vi "Ref Plots Viewer.vi"() -> ()   [LabVIEW 2020]
uses:
  Typedefs/Ref plot graphs cluster.ctl
  RIG-SPECIFIC FILES/FPGA Refs/FPGA Ref.ctl
  Movement Correction/Typedefs/Reference plots window ctrl refs.ctl
  Typedefs/Save-Load enum.ctl
  Typedefs/fgv_actions.ctl
  Typedefs/Read Write Enum.ctl
  templates/Queue Access FGV/Controls/FGV State Command.ctl
  Global Variables/General Globals.vi
  Globals/gl_Windows Ctrl refs.vi
  <vilib>/Utility/error.llb/Error Cluster From Error Code.vi
  <vilib>/rvi/errors/niLvFpgaAdjustHostInterfaceError.vi
  Global Variables/FPGAstatus_Reference.vi
  <vilib>/rvi/interface/nirviReadWriteControl/nirviReadWriteControl.xnode
  <vilib>/rvi/interface/Simulation/niFpgaSimulationCallBeginRW.vi
  NiFpgaLv.dll
panel:
  in  "Auto reset":bool
  out "Actual refresh rate (ms)":u32
  in  "Initiate reset":bool
  in  "Lower limits [um]":dbl=-115.0
  in  "Upper limits [um]":dbl=115.0
  out "L1 Time":u32
  out "L2 Time":u32
  out "# pending insert":i32
  out "# pending remove":i32
  out "RESTART MC":bool
  out "Reset Transition Status":T1(ring)
  out "Status":T2(ring)
  out "Graph Updating":bool
  in  "Ref image thresholding":cluster{"Numeric":dbl, "Numeric":dbl}(slide)={"Numeric"=0.0, "Numeric"=819.0} scale=0.0..4095.0
  out "Test GraphData Path":path
  in  "Append Date-Time":bool
  in  "Append file name":string
  out "MC Data Save ON":bool
  in  "Save MC Data":bool
  in  "Nth Frame":u16=11 min=10 step=10
  out "end of trial":i16(graph)
  in  "Frames":i16=1
  out "FPGA VI Reference Out":T3
  in  "Maximum Value":i32=4095
  in  "Minimum Value":i32
  out "Ref Image":T4(plugin-control)
  out "background_mc":bool
  out "bgsm_state":T5(ring)
  out "Acquire MC BG":bool
  out "rec_on_bg":bool
  out "aq state":T6(ring)
  in  "Acquisition completed":bool
  out "Stop (ind)":bool
  out "error":errorcluster
  in  "Snapshot file path":path caption="Snapshot file path (data is appended if same file used)"
  in  "Buffer Size":i32=5000 min=5 max=10000 step=100
  in  "Refresh rate (ms)":u32=500 min=10 step=10
  in  "Snapshot":bool
  in  "Reset Graphs":bool
  out "Graphs cluster":T7
  # "(during live imaging)"
  # "12"
  # "2"
  # "0"
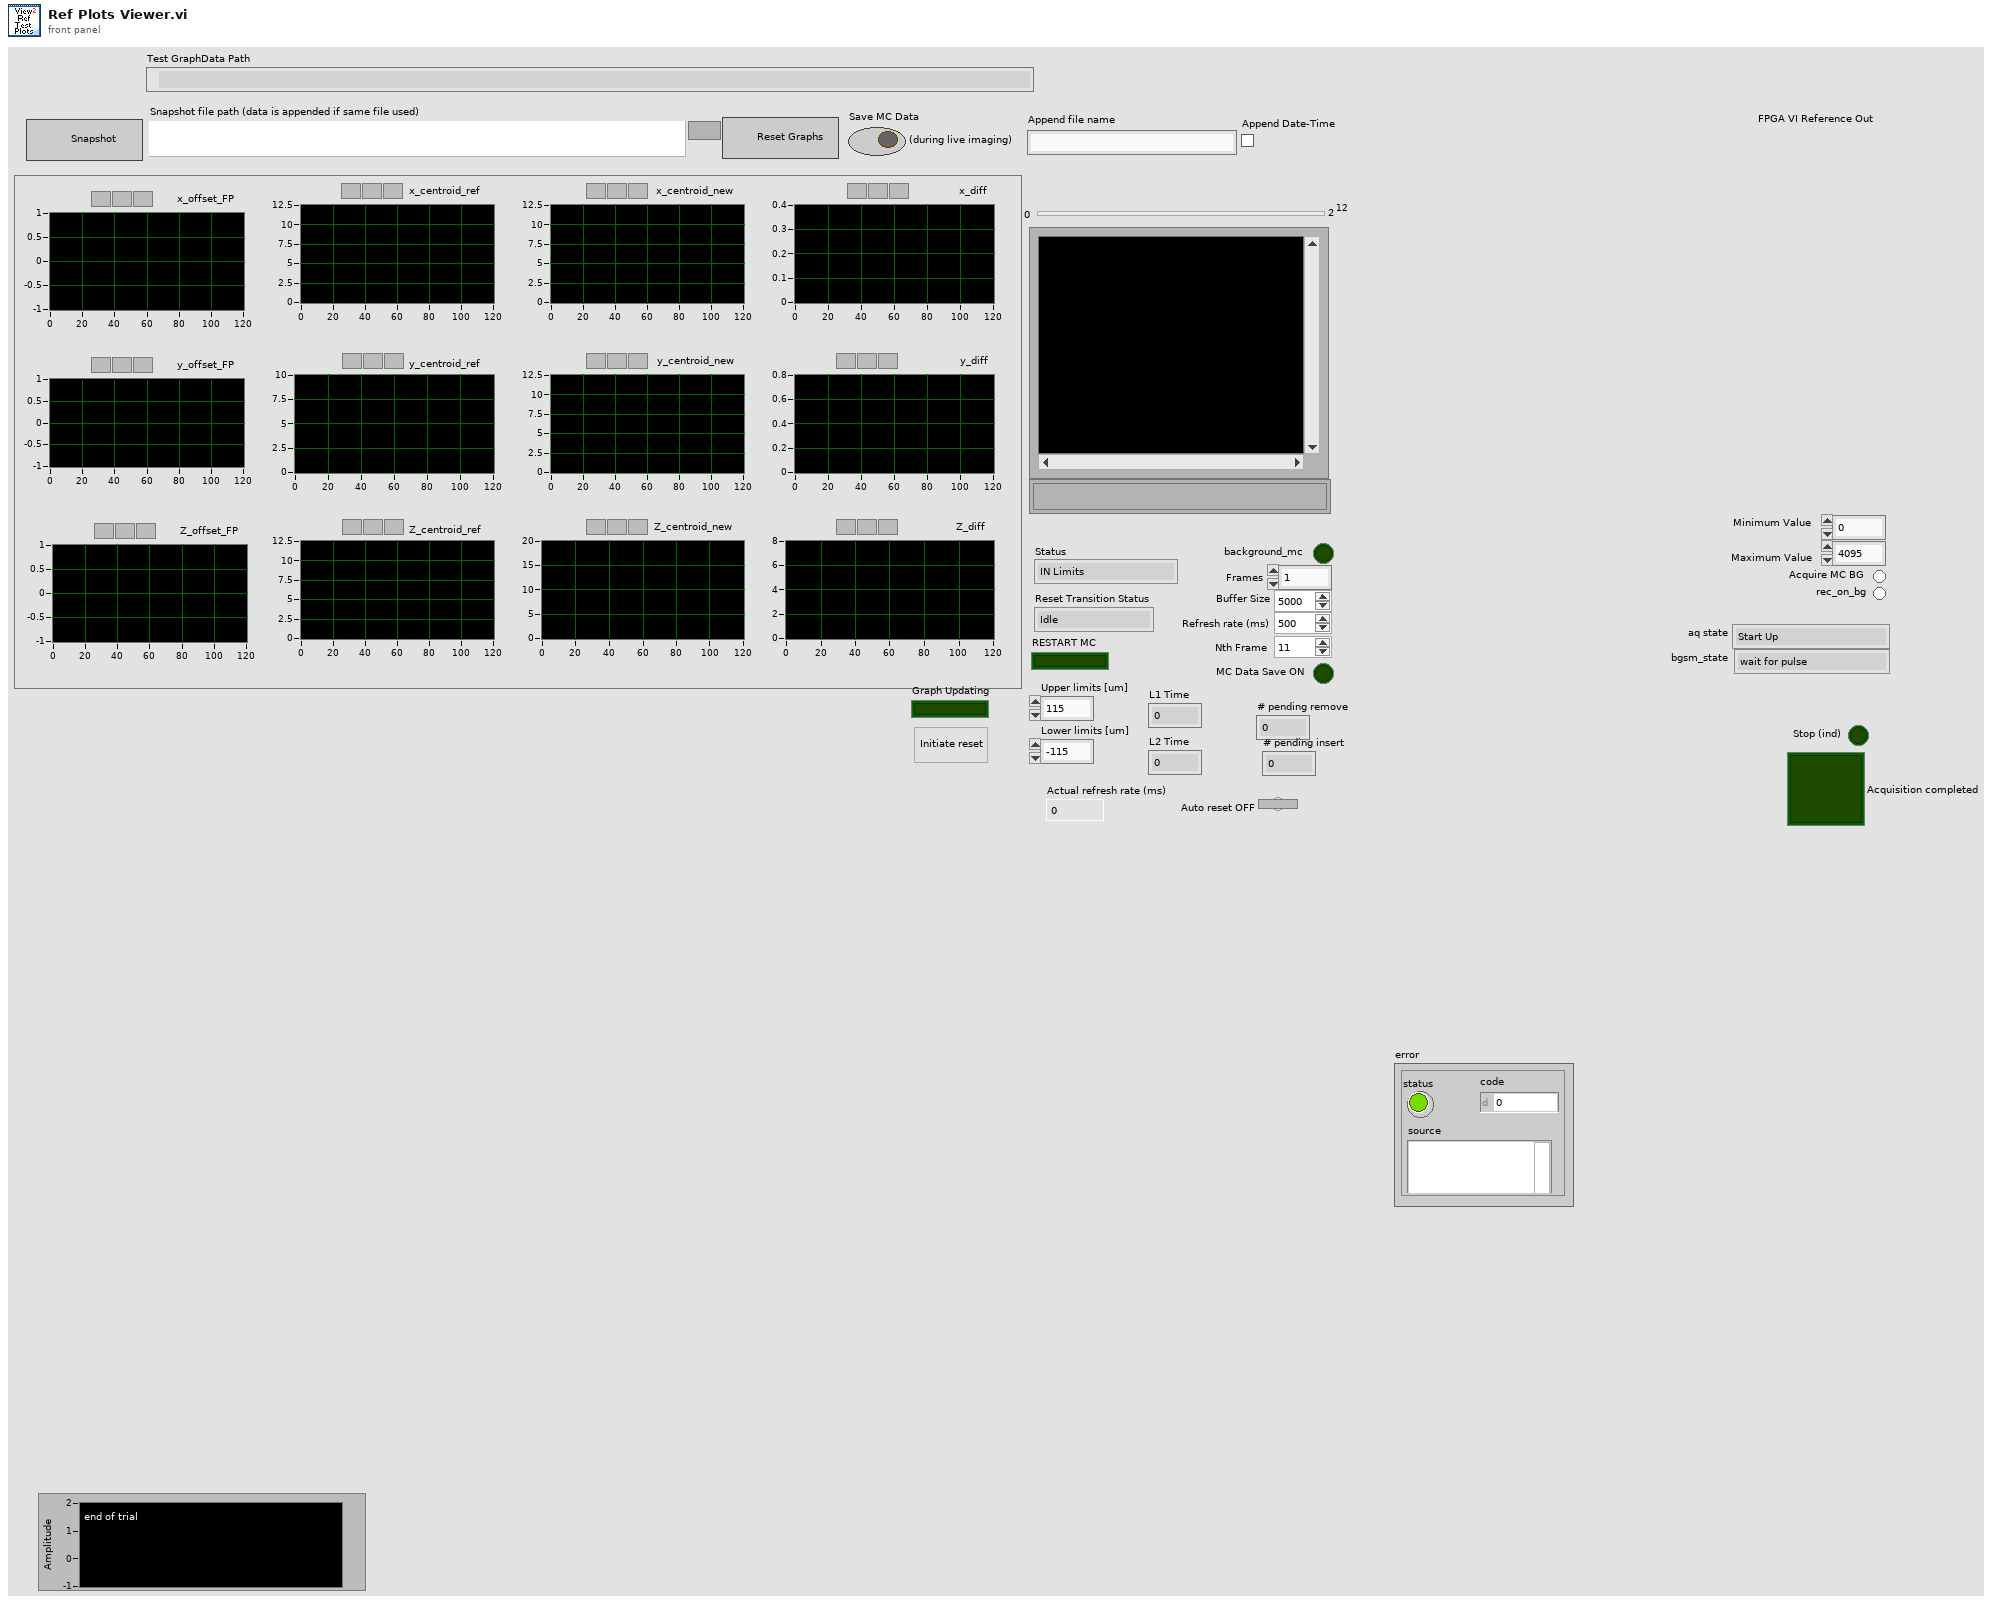
[diagram p1: front panel]
types:
  T1 = enum16{"Idle", "Stop MC Tracking", "Wait process", "Monitor error", "Restart MC Tracking"}
  T2 = enum16{"IN Limits", "X/Y Exceeded", "Z Exceeded", "X/Y & Z Exceeded"}
  T3 = typedef "FPGA Ref.ctl" = refnum<k20>
  T4 = typedef "IMAQ Image.ctl" = refnum<image>
  T5 = enum16{"wait for pulse", "wiat for N after pulse", "refernce frame", "ref aod fill bg"}
  T6 = enum16{"Start Up", "Wait for Trigger", "Wait N after Trigger", "DAQ Pointing", "DAQ Scan", "Reference Scan", "Pointing AOL Fill", "Scan AOL FILL", "Reference AOL Fill"}
  T7 = typedef "Ref plot graphs cluster.ctl" = cluster{"x_offset_FP":dbl[], "y_offset_FP":dbl[], "x_centroid_ref":dbl[], "y_centroid_ref":dbl[], "x_centroid_new":dbl[], "y_centroid_new":dbl[], "x_diff":dbl[], "y_diff":dbl[], "Z_offset_FP":dbl[], "Z_centroid_ref":dbl[], "Z_centroid_new":dbl[], "Z_diff":dbl[]}
  T8 = typedef "Image Type" = u32
  T9 = typedef "Reference plots window ctrl refs.ctl" = cluster{"Refresh rate (ms)":refnum<vi>, "Buffer Size":refnum<vi>}
  T10 = typedef "Save-Load enum.ctl" = enum16{"Save to file", "Load from file", "Compare from file", "Save Backup"}
  T11 = enum16{"Obtain queue", "Call window", "Call & send signal", "Release queue"}
  T12 = typedef "fgv_actions.ctl" = enum16{"Get", "Set"}
  T13 = typedef "Read Write Enum.ctl" = enum16{"Read", "Write"}
  T14 = typedef "FGV State Command.ctl" = enum16{"Get", "Initialize", "Release"}
  T15 = enum16{"Start Up", "Wait for Trigger", "Wait N after Trigger", "DAQ Pointing", "DAQ Scan", "Reference Scan", "Pointing AOL Fill", "Scan AOL FILL", "Reference AOL Fill", "galvo_moving", "wait_extra_ref"}
  T16 = cluster{"Conversion Method":u32, "Minimum Value":i32, "Maximum Value":i32, "Number Of Shifts":i32}
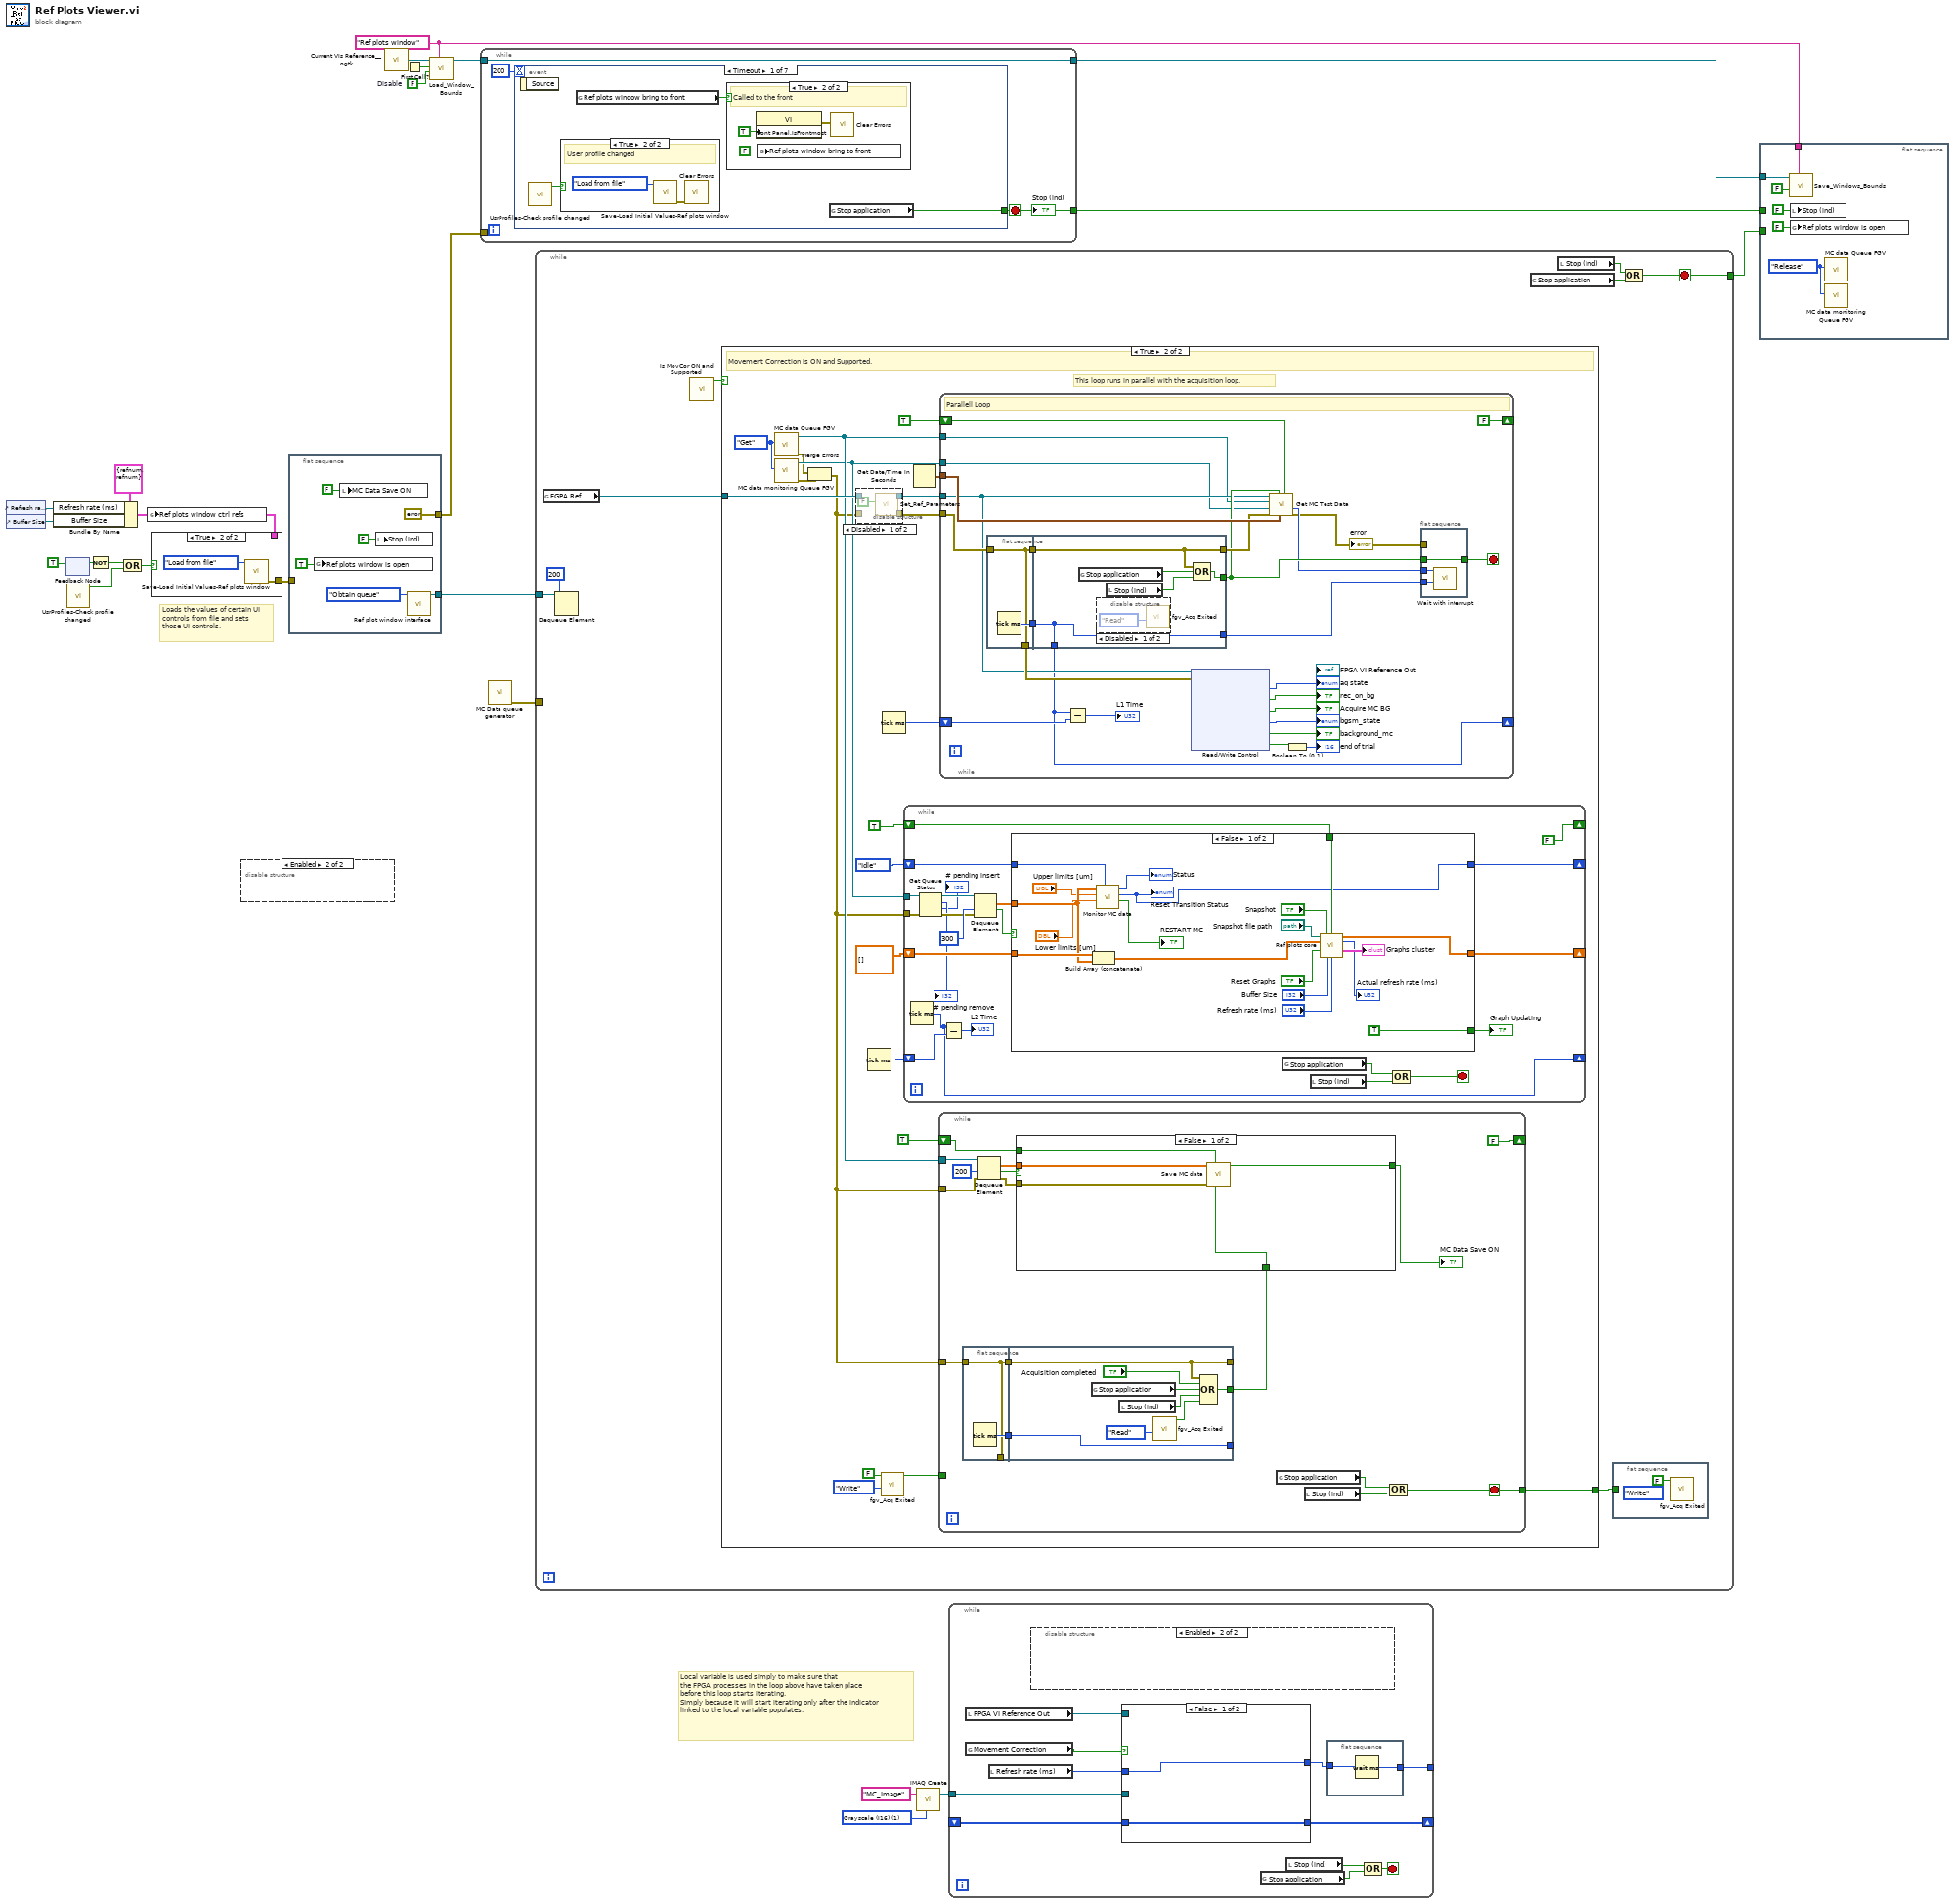
[diagram p0: block diagram]
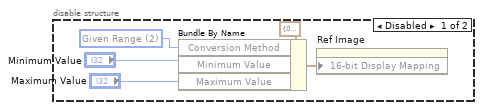
[diagram p2: hidden frame]
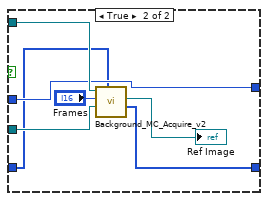
[diagram p3: hidden frame]
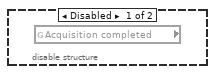
[diagram p4: hidden frame]
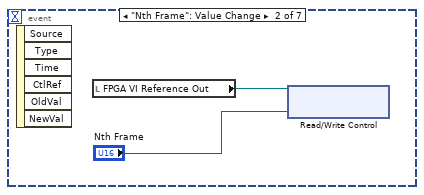
[diagram p8: hidden frame]
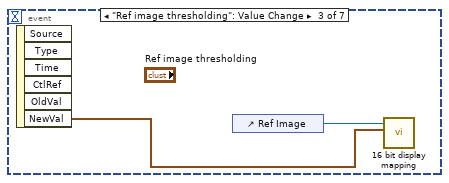
[diagram p9: hidden frame]
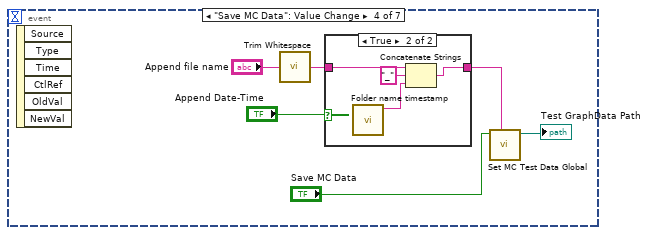
[diagram p10: hidden frame]
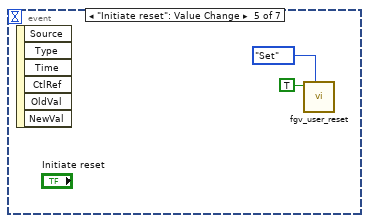
[diagram p12: hidden frame]
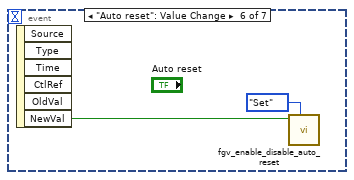
[diagram p13: hidden frame]
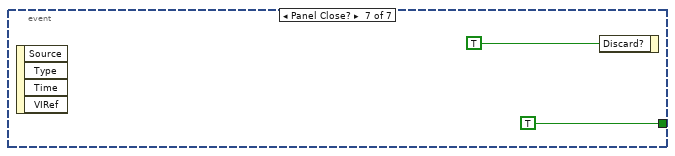
[diagram p14: hidden frame]
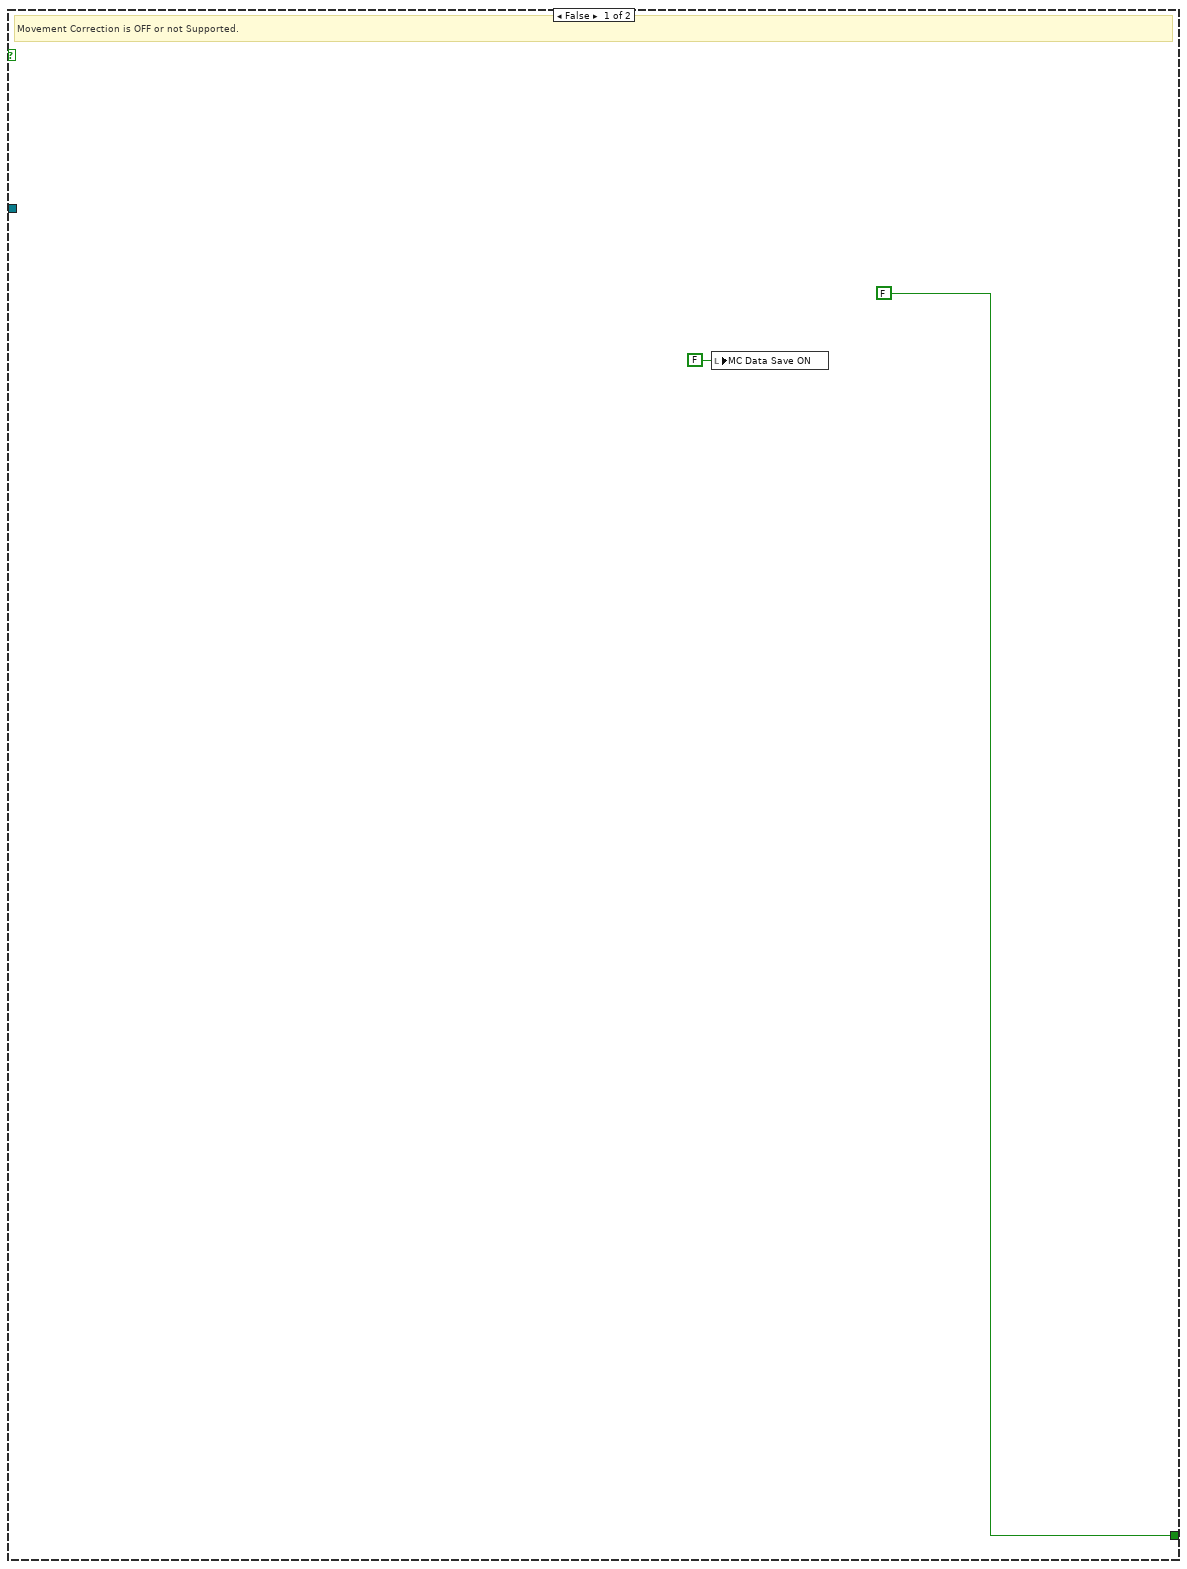
[diagram p15: hidden frame]
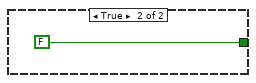
[diagram p16: hidden frame]
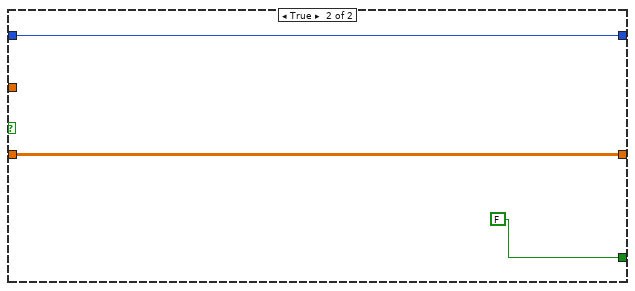
[diagram p17: hidden frame]
diagram:
  w3 = T8 1 items=["Grayscale (U8)", "Grayscale (I16)", "Grayscale (SGL)", "Complex (CSG)", "RGB (U32)", "HSL (U32)", "RGB (U64)", "Grayscale (U16)"] ("Image Type")
  w19 = FALSE  # Disable
  w7 = "Ref plots window" ("Window Name (i.e. Key)")
  # "Local variable is used simply to make sure that\nthe FPGA processes in the loop above have taken place\nbefore this loop starts iterating.\nSImply because it will start iterating only after the indicator\nlinked to the local variable populates."
  # "Loads the values of certain UI controls from file and sets those UI controls."
  n1 = control-ref of="Refresh rate (ms)"() -> (w14:refnum<vi>)
  n2 = control-ref of="Buffer Size"() -> (w13:refnum<vi>)
  n3 = Bundle By Name(cluster=T9 {"Refresh rate (ms)"=refnum, "Buffer Size"=refnum} ("Reference plots window ctrl refs"), "Refresh rate (ms)"=w14, "Buffer Size"=w13) -> (w15:T9)
  n4 = feedback #1() -> (w12:bool)  [unwired: 1 in]
  n5 = feedback-in #1(TRUE) -> ()
  n6 = call "UsrProfiles-Check profile changed.vi"() -> ("Profile changed"=w9:bool)  [unwired: 10 in, 1 out]
  n7 = Not(x=w12) -> (.not. x?=w10:bool)
  n8 = Compound Arithmetic op=OR(w10, w9) -> (w8:bool)
  n9 = global write "gl_Windows Ctrl refs.vi" "Ref plots window ctrl refs"(w15) -> ()
  n10 = case shown="True" w8 {
    tunnel: [_ w25] -> w17
    tunnel: w15 -> [_ _]
    frame False {
    }
    frame True {
      n11 = call "Save-Load Initial Values-Ref plots window.vi"("Function"=Save-Load_enum."Load from file") -> ("error out"=w25:errorcluster)  [unwired: 10 in]
    }
  }
  n12 = disable-structure shown="Enabled" {
    frame Disabled {
      n13 = global read "General Globals.vi" "Acquisition completed"() -> ()  [unwired: 1 out]
    }
    frame Enabled {
    }
  }
  n14 = flat-sequence {
    tunnel: [w31] -> w24
    tunnel: [errorcluster {"status"=FALSE, "code"=0, "source"=""} ("error out")] -> w22
    tunnel: w17 -> [_]
    frame #0 {
      n15 = global write "General Globals.vi" "Ref plots window is open"(TRUE ("Ref plots window is open")) -> ()
      n16 = local write "MC Data Save ON"(FALSE ("MC Data Save ON")) -> ()
      n17 = local write "Stop (ind)"(FALSE ("Stop (ind)")) -> ()
      n18 = call "Ref plot window interface.vi"("Function"=T11."Obtain queue") -> ("Ref plots window queue"=w31:refnum<queue>)  [unwired: 9 in, 1 out]
    }
  }
  n19 = call <userlib>:"Current VIs Reference__ogtk.vi"() -> ("Current VI's reference"=w21:refnum<vi>)  [unwired: 5 in]
  n20 = First Call?() -> (First Call?: T/F=w20:bool)
  n21 = call "Load_Window_Bounds.vi"("Window Name (i.e. Key)"=w7, "Disable"=w19, "First Call"=w20, "Window VI's Ref"=w21) -> ("reference out"=w18:refnum<vi>)  [unwired: 4 in, 3 out]
  n22 = while {
    tunnel: [w33] -> w5
    tunnel: w22 -> [_]
    tunnel: w18 -> [w34]
    tunnel: [w34] -> w6
    stop <- w33 stop-if-true
    n23 = event shown="[0] Timeout" {
      selector: _ -> [_ _ _ _ _ _ _]
      dyn-events: _ -> [_ _ _ _ _ _ _]
      timeout: 200 -> [_ _ _ _ _ _ _]
      tunnel: [w38 _ _ _ _ _ TRUE ("Stop application")] -> w33
      event Timeout {
        n24 = event-data() -> ()  [unwired: 1 in, 1 out]
        n25 = call "UsrProfiles-Check profile changed.vi"() -> ("Profile changed"=w36:bool)  [unwired: 10 in, 1 out]
        n26 = case shown="True" w36 {
          frame False {
            # "Idle"
          }
          frame True {
            # "User profile changed"
            n27 = call "Save-Load Initial Values-Ref plots window.vi"("Function"=Save-Load_enum."Load from file") -> ("error out"=w39:errorcluster)  [unwired: 10 in]
            n28 = call <vilib>:"Clear Errors.vi"("error in (no error)"=w39) -> ()  [unwired: 5 in, 2 out]
          }
        }
        n29 = global read "General Globals.vi" "Ref plots window bring to front"() -> (w37:bool)
        n30 = case shown="True" w37 {
          frame False {
            # "Idle"
          }
          frame True {
            # "Called to the front"
            n31 = property class="VI"("Front Panel.IsFrontmost"=TRUE ("Front Panel Window:Is Frontmost")) -> (error out=w42:errorcluster)  [unwired: 2 in, 1 out]
            n32 = global write "General Globals.vi" "Ref plots window bring to front"(FALSE ("\"Funct img\" bring to front")) -> ()
            n33 = call <vilib>:"Clear Errors.vi"("error in (no error)"=w42) -> ()  [unwired: 5 in, 2 out]
          }
        }
        n34 = global read "General Globals.vi" "Stop application"() -> (w38:bool)
      }
      event "Nth Frame": Value Change {
        n35 = event-data() -> ()  [unwired: 1 in, 6 out]
        n36 = local read "FPGA VI Reference Out"() -> (w45:T3)
        n37 = xnode "Read/Write Control"("FPGA VI Reference In"=w45, "ref_frame dilute"="Nth Frame") -> ()  [unwired: 1 in, 2 out]
      }
      event "Ref image thresholding": Value Change {
        n38 = event-data() -> ("NewVal"=w46:cluster{"Numeric":dbl, "Numeric":dbl})  [unwired: 1 in, 5 out]
        n39 = control-ref of="Ref Image"() -> (w47:refnum<vi>)
        n40 = call "16 bit display mapping.vi"("16 bit display mapping"=w46, "Image Display"=w47) -> ()  [unwired: 8 in, 2 out]
      }
      event "Save MC Data": Value Change {
        n41 = event-data() -> ()  [unwired: 1 in, 6 out]
        n42 = call <vilib>:"Trim Whitespace.vi"("string"="Append file name") -> ("trimmed string"=w51:string)  [unwired: 1 in]
        n43 = case shown="True" "Append Date-Time" {
          tunnel: w51 -> [w54 w58]
          tunnel: [w54 w55] -> w50
          frame False {
          }
          frame True {
            n44 = call "Folder name timestamp.vi"() -> ("date/time string"=w56:string)  [unwired: 11 in]
            n45 = Concatenate Strings(w58, "_" ("string"), w56) -> (w55:string)
          }
        }
        n46 = call "Set MC Test Data Global.vi"("Append Name"=w50, "Save MC TestData"="Save MC Data") -> ("Test GraphData Path"=→"Test GraphData Path":path)  [unwired: 8 in, 1 out]
      }
      event "Initiate reset": Value Change {
        n47 = event-data() -> ()  [unwired: 1 in, 6 out]
        n48 = call "fgv_user_reset.vi"("FGV Actions"=fgv_actions."Set", "User reset"=TRUE) -> ()  [unwired: 8 in, 2 out]
      }
      event "Auto reset": Value Change {
        n49 = event-data() -> ("NewVal"=w61:bool)  [unwired: 1 in, 5 out]
        n50 = call "fgv_enable_disable_auto_reset.vi"("FGV Actions"=fgv_actions."Set", "Auto reset"=w61) -> ()  [unwired: 8 in, 2 out]
      }
      event Panel Close? {
        n51 = event-data() -> ()  [unwired: 1 in, 4 out]
        n52 = event-data("Discard?"=TRUE) -> ()  [unwired: 1 in, 1 out]
      }
    }
    "Stop (ind)" <- w33
  }
  n53 = call "MC Data queue generator.vi"() -> ("error out"=w1:errorcluster)  [unwired: 11 in]
  n54 = while {
    tunnel: [w69] -> w23
    tunnel: w24 -> [w71]
    tunnel: w1 -> [_]
    stop <- w69 stop-if-true
    n55 = global read "FPGAstatus_Reference.vi" "FGPA Ref"() -> (w67:T3)
    n56 = Dequeue Element(queue=w71, timeout in ms (-1)=200) -> ()  [unwired: 1 in, 4 out]
    n57 = call "Is MovCor ON and Supported.vi"() -> ("MovCor is ON and Supported"=w65:bool)  [unwired: 11 in]
    n58 = case shown="True" w65 {
      tunnel: [FALSE w82] -> w66
      tunnel: w67 -> [_ w90]
      frame False {
        # "Movement Correction is OFF or not Supported."
        n59 = local write "MC Data Save ON"(FALSE ("MC Data Save ON")) -> ()
      }
      frame True {
        w87 = FGV_State_Command."Get" ("FGV State Command")
        # "This loop runs in parallel with the acquisition loop."
        # "Movement Correction is ON and Supported."
        n60 = call "MC data Queue FGV.vi"("FGV State Command"=w87) -> ("queue out"=w86:refnum<queue>, "error out"=w83:errorcluster)  [unwired: 8 in]
        n61 = call "MC data monitoring Queue FGV.vi"("FGV State Command"=w87) -> ("queue out"=w85:refnum<queue>, "error out"=w84:errorcluster)  [unwired: 8 in]
        n62 = Merge Errors(w83, w84) -> (w78:errorcluster)
        n63 = disable-structure shown="Disabled" {
          disable-tunnel: [w173 w175] -> w95
          disable-tunnel: [w172 w176] -> w80
          disable-tunnel: w90 -> [_ w176]
          disable-tunnel: w78 -> [_ w175]
          frame Disabled {
            n64 = call "Set_Ref_Parameters.vi"("use_increment_halfrate"=FALSE) -> ("error out"=w173:errorcluster, "FPGA VI Reference Out"=w172:T3)  [unwired: 8 in, 1 out]
          }
          frame Enabled {
          }
        }
        n65 = Tick Count (ms)() -> (millisecond timer value=w77:u32)
        n66 = call "fgv_Acq Exited.vi"("Function"=Read_Write_Enum."Write", "Acquisition completed"=FALSE ("Timelapse?")) -> ("Acquisition completed"=w81:bool)  [unwired: 8 in, 1 out]
        n67 = Tick Count (ms)() -> (millisecond timer value=w76:u32)
        n68 = while {
          shift-right: [FALSE] -> _
          shift-left: TRUE -> [w141]
          tunnel: w85 -> [w138]
          tunnel: w78 -> [w137]
          shift-right: [w140] -> _
          shift-left: dbl[][] [] -> [w142]
          shift-right: [w130] -> _
          shift-left: w77 -> [w132]
          shift-right: [w128] -> _
          shift-left: T1."Idle" ("IP/condition") -> [w129]
          stop <- w147 stop-if-true
          n69 = Tick Count (ms)() -> (millisecond timer value=w130:u32)
          n70 = Get Queue Status(queue=w138, error in (no error)=w137) -> (queue out=w136:refnum<queue>, # pending remove=→"# pending remove":i32, # pending insert=→"# pending insert":i32, error out=w135:errorcluster)  [unwired: 1 in, 4 out]
          n71 = Subtract(x=w130, y=w132) -> (x-y=→"L2 Time":u32)
          n72 = Dequeue Element(queue=w136, timeout in ms (-1)=300, error in (no error)=w135) -> (element=w143:dbl[], timed out?=w144:bool)  [unwired: 2 out]
          n73 = case shown="False" w144 {
            tunnel: w143 -> [w158 _]
            tunnel: w142 -> [w168 w171]
            tunnel: w141 -> [w161 _]
            tunnel: [w155 w171] -> w140
            tunnel: [TRUE FALSE] -> w139
            tunnel: w129 -> [w152 w169]
            tunnel: [w151 w169] -> w128
            frame False {
              n74 = Build Array (concatenate)(w168, w158) -> (w160:dbl[][])
              n75 = call "Monitor MC data.vi"("IP/condition"=w152, "Lower limits [um]"="Lower limits [um]", "Upper limits [um]"="Upper limits [um]", "MC data IN"=w158) -> ("RESTART MC"=→"RESTART MC":bool, "Reset Transition Status"=w151:T1, "Status"=→"Status":T2)  [unwired: 4 in, 1 out]
              "Reset Transition Status" <- w151
              n76 = call "Ref plots core.vi"("Snapshot file path"="Snapshot file path", "Snapshot"="Snapshot", "Initialise"=w161, "Ref Test Data in in"=w160, "Reset Graphs"="Reset Graphs", "Buffer Size"="Buffer Size", "Refresh rate (ms)"="Refresh rate (ms)") -> ("Ref Test Data out"=w155:dbl[][], "Actual refresh rate (ms)"=→"Actual refresh rate (ms)":u32, "Graphs cluster"=→"Graphs cluster":T7)  [unwired: 5 in, 1 out]
            }
            frame True {
            }
          }
          "Graph Updating" <- w139
          n77 = global read "General Globals.vi" "Stop application"() -> (w149:bool)
          n78 = local read "Stop (ind)"() -> (w148:bool)
          n79 = Compound Arithmetic op=OR(w149, w148) -> (w147:bool)
        }
        n80 = Get Date/Time In Seconds() -> (seconds since 1Jan1904=w94:timestamp)
        n81 = while {
          shift-right: [FALSE] -> _
          shift-left: TRUE -> [w101]
          tunnel: w86 -> [w107]
          tunnel: w78 -> [w109]
          tunnel: [w97] -> w82
          tunnel: w81 -> [_]
          tunnel: w78 -> [w106]
          stop <- w97 stop-if-true
          n82 = flat-sequence {
            tunnel: [w119] -> w111
            tunnel: [w118] -> w110
            tunnel: w109 -> [w118]
            tunnel: [w118] -> _
            tunnel: [w125] -> w100
            tunnel: [w124] -> _
            tunnel: w111 -> [w124]
            tunnel: w110 -> [w123]
            tunnel: [w123] -> _
            frame #0 {
              n83 = Tick Count (ms)() -> (millisecond timer value=w119:u32)
            }
            frame #1 {
              n84 = global read "General Globals.vi" "Stop application"() -> (w127:bool)
              n85 = local read "Stop (ind)"() -> (w121:bool)
              n86 = call "fgv_Acq Exited.vi"("Function"=Read_Write_Enum."Read") -> ("Acquisition completed"=w122:bool)  [unwired: 9 in, 1 out]
              n87 = Compound Arithmetic op=OR(w123, "Acquisition completed", w127, w121, w122) -> (w125:bool)
            }
          }
          n88 = Dequeue Element(queue=w107, timeout in ms (-1)=200, error in (no error)=w106) -> (element=w105:dbl[], timed out?=w102:bool, error out=w103:errorcluster)  [unwired: 1 out]
          n89 = case shown="False" w102 {
            tunnel: w105 -> [w116 _]
            tunnel: w103 -> [w115 _]
            tunnel: w101 -> [w114 _]
            tunnel: [w113 FALSE ("MC Data Save ON")] -> w96
            tunnel: w100 -> [w112 _]
            frame False {
              n90 = call "Save MC data.vi"("Stop"=w112, "Initialise"=w114, "error in (no error)"=w115, "Input"=w116) -> ("MC Data Save ON"=w113:bool)  [unwired: 6 in, 1 out]
            }
            frame True {
            }
          }
          "MC Data Save ON" <- w96
          n91 = global read "General Globals.vi" "Stop application"() -> (w98:bool)
          n92 = local read "Stop (ind)"() -> (w99:bool)
          n93 = Compound Arithmetic op=OR(w98, w99) -> (w97:bool)
        }
        n94 = while {
          tunnel: w80 -> [w187]
          tunnel: w95 -> [w197]
          tunnel: w94 -> [w202]
          shift-right: [FALSE] -> _
          shift-left: TRUE -> [w193]
          tunnel: w86 -> [w182]
          tunnel: w85 -> [w181]
          shift-right: [w177] -> _
          shift-left: w76 -> [w179]
          stop <- w201 stop-if-true
          # "Parallell Loop"
          n95 = flat-sequence {
            tunnel: [w205] -> w199
            tunnel: [w204] -> w198
            tunnel: w197 -> [w204]
            tunnel: [w204] -> w188
            tunnel: [w209] -> w195
            tunnel: [w206] -> w200
            tunnel: w199 -> [w206]
            tunnel: w198 -> [w208]
            tunnel: [w208] -> w196
            tunnel: [w206] -> w177
            frame #0 {
              n96 = Tick Count (ms)() -> (millisecond timer value=w205:u32)
            }
            frame #1 {
              n97 = global read "General Globals.vi" "Stop application"() -> (w210:bool)
              n98 = disable-structure shown="Disabled" {
                frame Disabled {
                  n99 = call "fgv_Acq Exited.vi"("Function"=Read_Write_Enum."Read") -> ()  [unwired: 9 in, 2 out]
                }
                frame Enabled {
                }
              }
              n100 = local read "Stop (ind)"() -> (w207:bool)
              n101 = Compound Arithmetic op=OR(w208, w210, w207) -> (w209:bool)
            }
          }
          n102 = Subtract(x=w177, y=w179) -> (x-y=→"L1 Time":u32)
          n103 = xnode ("Read/Write Control")("FPGA VI Reference In"=w187, "error in"=w188) -> ("FPGA VI Reference Out"=→"FPGA VI Reference Out":T3, "aq state"=→"aq state":T15, "rec_on_bg"=→"rec_on_bg":bool, "Acquire MC BG"=→"Acquire MC BG":bool, "bgsm_state"=→"bgsm_state":T5, "background_mc"=→"background_mc":bool, "end of trial"=w183:bool)  [unwired: 1 out]
          n104 = call "Get MC Test Data.vi"("Initialise"=w193, "Initial Time Stamp"=w202, "Stop"=w195, "error in (no error)"=w196, "MC Data montoring queue IN"=w181, "MC Data queue IN"=w182, "FPGA Ref in"=w187) -> ("error out"=w180:errorcluster, "MC state"=w194:enum16{"Waiting", "First frame", "Wrote Ref"})  [unwired: 3 in]
          "error" <- w180
          n105 = Boolean To (0,1)(Boolean=w183) -> (0, 1=→"end of trial":i16)
          n106 = flat-sequence {
            tunnel: w195 -> [w214]
            tunnel: [w214] -> w201
            tunnel: w200 -> [w213]
            tunnel: w194 -> [w212]
            tunnel: w180 -> [_]
            frame #0 {
              n107 = call "Wait with interrupt.vi"("Tick count at loop start (ms)"=w213, "Loop iteration (ms)"=w212) -> ()  [unwired: 10 in]
            }
          }
        }
      }
    }
    n108 = global read "General Globals.vi" "Stop application"() -> (w72:bool)
    n109 = local read "Stop (ind)"() -> (w68:bool)
    n110 = flat-sequence {
      tunnel: w66 -> [_]
      frame #0 {
        n111 = call "fgv_Acq Exited.vi"("Function"=Read_Write_Enum."Write", "Acquisition completed"=FALSE ("Timelapse?")) -> ()  [unwired: 8 in, 2 out]
      }
    }
    n112 = Compound Arithmetic op=OR(w68, w72) -> (w69:bool)
  }
  n113 = call "IMAQ Create"("Image Name"="MC_Image", "Image Type"=w3) -> ("New Image"=w2:T4)  [unwired: 3 in, 1 out]
  n114 = while {
    tunnel: w2 -> [w224]
    tunnel: [w220] -> _
    shift-right: [w218] -> _
    shift-left: _ -> [w217]
    stop <- w225 stop-if-true
    n115 = local read "FPGA VI Reference Out"() -> (w223:T3)
    n116 = global read "General Globals.vi" "Movement Correction"() -> (w219:bool)
    n117 = local read "Refresh rate (ms)"() -> (w222:u32)
    n118 = disable-structure shown="Enabled" {
      frame Disabled {
        w228 = u32 2 items=["Full Dynamic", "Downshift", "Given Range", "90% Dynamic", "Given Percent Range"] ("Conversion Method (Given Range)")
        n119 = Bundle By Name(cluster=T16 {"Conversion Method"=0, "Minimum Value"=0, "Maximum Value"=0, "Number Of Shifts"=0} ("16-bit Display Mapping:All Elements"), "Conversion Method"=w228, "Minimum Value"="Minimum Value", "Maximum Value"="Maximum Value") -> (w230:T16)
        n120 = property on="Ref Image" class="ImageControl"("16-bit Display Mapping"=w230) -> ()  [unwired: 2 in, 2 out]
      }
      frame Enabled {
      }
    }
    n121 = case shown="False" w219 {
      tunnel: w223 -> [_ w243]
      tunnel: w224 -> [_ w242]
      tunnel: w222 -> [w236 w239]
      tunnel: [w236 w239] -> w221
      tunnel: [w235 w238] -> w218
      tunnel: w217 -> [w235 w237]
      frame False {
      }
      frame True {
        n122 = call "Background_MC_Acquire_v2.vi"("prev deleted portion"=w237, "Image In"=w242, "Frames"="Frames", "FPGA VI Reference In"=w243) -> ("deleted portion"=w238:u16[], "Image"=→"Ref Image":T4)  [unwired: 4 in, 2 out]
      }
    }
    n123 = global read "General Globals.vi" "Stop application"() -> (w226:bool)
    n124 = local read "Stop (ind)"() -> (w227:bool)
    n125 = flat-sequence {
      tunnel: [w234] -> w220
      tunnel: w221 -> [w233]
      frame #0 {
        n126 = Wait (ms)(milliseconds to wait=w233) -> (millisecond timer value=w234:u32)
      }
    }
    n127 = Compound Arithmetic op=OR(w227, w226) -> (w225:bool)
  }
  n128 = flat-sequence {
    tunnel: w23 -> [_]
    tunnel: w7 -> [w246]
    tunnel: w6 -> [w245]
    tunnel: w5 -> [_]
    frame #0 {
      w244 = FGV_State_Command."Release" ("FGV State Command")
      n129 = call "Save_Windows_Bounds.vi"("Window Name (i.e. Key)"=w246, "Front Panel Window:Open"=FALSE, "Window VI's Ref"=w245) -> ()  [unwired: 8 in, 1 out]
      n130 = local write "Stop (ind)"(FALSE ("Stop (ind)")) -> ()
      n131 = global write "General Globals.vi" "Ref plots window is open"(FALSE ("Ref plots window is open")) -> ()
      n132 = call "MC data Queue FGV.vi"("FGV State Command"=w244) -> ()  [unwired: 8 in, 2 out]
      n133 = call "MC data monitoring Queue FGV.vi"("FGV State Command"=w244) -> ()  [unwired: 8 in, 2 out]
    }
  }
